vi "循环扫描脚本.vi"(8 "4-wire":bool, 11 "扫描参数":T1={"+ V"=1.0, "+ Δ V"=0.01, "+ limit I"=0.01, "- V"=1.0, "- Δ V"=0.01, "- limit I"=0.01, "NPLC"=1.0, "模型"=FALSE} {"NPLC" min=0.001 max=25.0 step=0.001; "- Δ V" min=5e-05 max=1.0 step=5e-05 format="%#_6pV"; "+ Δ V" min=5e-05 max=1.0 step=5e-05 format="%#_6pV"; "- V" min=-40.0 max=40.0 format="%#_6pV"; "- limit I" min=1e-08 max=3.0 format="%#_6pA"; "+ limit I" min=1e-08 max=3.0 format="%#_6pA"; "+ V" min=-40.0 max=40.0 format="%#_6pV"}) -> (3 "Script":string)   [LabVIEW 2020, in "功能选择.xctl"]
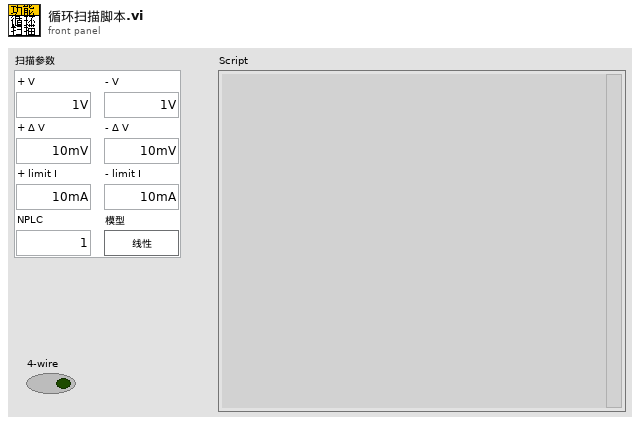
[diagram p1: front panel]
types:
  T1 = typedef "功能选择.xctl/扫描参数.ctl" = cluster{"+ V":dbl, "+ Δ V":dbl, "+ limit I":dbl, "- V":dbl, "- Δ V":dbl, "- limit I":dbl, "NPLC":dbl, "模型":bool}
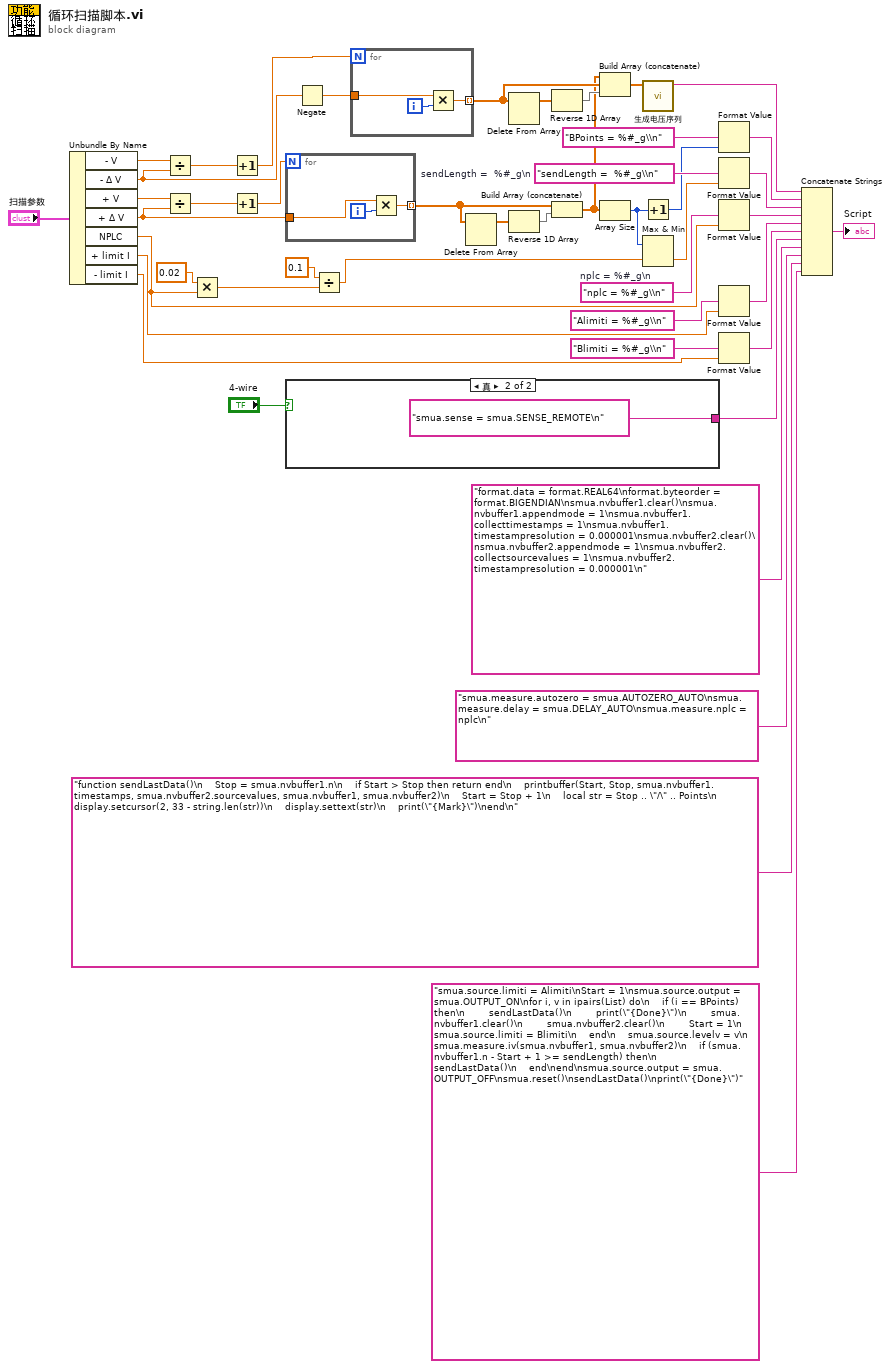
[diagram p0: block diagram]
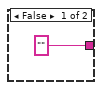
[diagram p2: hidden frame]
diagram:
  w34 = "nplc = %#_g\\n"  # nplc = %#_g\n
  w43 = "sendLength =  %#_g\\n"  # sendLength =  %#_g\n
  n1 = Unbundle By Name("扫描参数") -> ("- V"=w15:dbl, "- Δ V"=w14:dbl, "+ V"=w42:dbl, "+ Δ V"=w40:dbl, "NPLC"=w16:dbl, "+ limit I"=w11:dbl, "- limit I"=w10:dbl)
  n2 = Divide(x=w15, y=w14) -> (x/y=w22:dbl)
  n3 = Divide(x=w42, y=w40) -> (x/y=w41:dbl)
  n4 = Multiply(x=0.02 ("y"), y=w16) -> (x*y=w32:dbl)
  n5 = Increment(x=w22) -> (x+1=w25:dbl)
  n6 = Increment(x=w41) -> (x+1=w37:dbl)
  n7 = for {
    N: w37 -> [_]
    tunnel: w40 -> [w48]
    tunnel: [w47] -> w36 mode=indexing
    i -> [w49]
    n8 = Multiply(x=w48, y=w49) -> (x*y=w47:dbl)
  }
  n9 = case shown="真" "4-wire" {
    tunnel: ["" "smua.sense = smua.SENSE_REMOTE\n"] -> w3
    frame False {
    }
    frame True {
    }
  }
  n10 = Negate(x=w14) -> (-x=w4:dbl)
  n11 = Divide(x=0.1, y=w32) -> (x/y=w31:dbl)
  n12 = for {
    N: w25 -> [_]
    tunnel: w4 -> [w53]
    tunnel: [w52] -> w26 mode=indexing
    i -> [w54]
    n13 = Multiply(x=w53, y=w54) -> (x*y=w52:dbl)
  }
  n14 = Delete From Array(array=w36) -> (array with subset deleted=w38:dbl[])  [unwired: 2 in, 1 out]
  n15 = Delete From Array(array=w26) -> (array with subset deleted=w24:dbl[])  [unwired: 2 in, 1 out]
  n16 = Reverse 1D Array(array=w38) -> (reversed array=w39:dbl[])
  n17 = Reverse 1D Array(array=w24) -> (reversed array=w23:dbl[])
  n18 = Build Array (concatenate)(w36, w39) -> (w19:dbl[])
  n19 = Build Array (concatenate)(w19, w26, w23) -> (w18:dbl[])
  n20 = Array Size(array=w19) -> (size(s)=w21:i32)
  n21 = call "生成电压序列.vi"("电压序列"=w18) -> ("List"=w6:string)  [unwired: 10 in]
  n22 = Increment(x=w21) -> (x+1=w20:i32)
  n23 = Max & Min(x=w21, y=w31) -> (min(x,y)=w30:dbl)  [unwired: 1 out]
  n24 = Format Value(format string="BPoints = %#_g\\n" ("格式字符串"), value (0)=w20) -> (output string=w7:string)  [unwired: 1 in]
  n25 = Format Value(format string=w43, value (0)=w30) -> (output string=w8:string)  [unwired: 1 in]
  n26 = Format Value(format string=w34, value (0)=w16) -> (output string=w9:string)  [unwired: 1 in]
  n27 = Format Value(format string="Alimiti = %#_g\\n" ("格式字符串"), value (0)=w11) -> (output string=w12:string)  [unwired: 1 in]
  n28 = Format Value(format string="Blimiti = %#_g\\n" ("格式字符串"), value (0)=w10) -> (output string=w13:string)  [unwired: 1 in]
  n29 = Concatenate Strings(w6, w7, w8, w9, w12, w13, w3, "format.data = format.REAL64\nformat.byteorder = format.BIGENDIAN\nsmua.nvbuffer1.clear()\nsmua.nvbuffer1.appendmode = 1\nsmua.nvbuffer1.collecttimestamps = 1\nsmua.nvbuffer1.timestampresolution = 0.000001\nsmua.nvbuffer2.clear()\nsmua.nvbuffer2.appendmode = 1\nsmua.nvbuffer2.collectsourcevalues = 1\nsmua.nvbuffer2.timestampresolution = 0.000001\n", "smua.measure.autozero = smua.AUTOZERO_AUTO\nsmua.measure.delay = smua.DELAY_AUTO\nsmua.measure.nplc = nplc\n", "function sendLastData()\n    Stop = smua.nvbuffer1.n\n    if Start > Stop then return end\n    printbuffer(Start, Stop, smua.nvbuffer1.timestamps, smua.nvbuffer2.sourcevalues, smua.nvbuffer1, smua.nvbuffer2)\n    Start = Stop + 1\n    local str = Stop .. \"/\" .. Points\n    display.setcursor(2, 33 - string.len(str))\n    display.settext(str)\n    print(\"{Mark}\")\nend\n", "smua.source.limiti = Alimiti\nStart = 1\nsmua.source.output = smua.OUTPUT_ON\nfor i, v in ipairs(List) do\n    if (i == BPoints) then\n        sendLastData()\n        print(\"{Done}\")\n        smua.nvbuffer1.clear()\n        smua.nvbuffer2.clear()\n        Start = 1\n        smua.source.limiti = Blimiti\n    end\n    smua.source.levelv = v\n    smua.measure.iv(smua.nvbuffer1, smua.nvbuffer2)\n    if (smua.nvbuffer1.n - Start + 1 >= sendLength) then\n        sendLastData()\n    end\nend\nsmua.source.output = smua.OUTPUT_OFF\nsmua.reset()\nsendLastData()\nprint(\"{Done}\")") -> (→"Script":string)
